vi "Open Deployed Project.vi"() -> ()   [LabVIEW 2023]
doc: "Tools >> Systemcore >> Open Deployed Project: copies the program a robot runs (its current deploy) into a git working copy on the robot-edits branch and opens its LabVIEW project. When the robot keeps several projects, the user chooses one. In the robot's own IDE it uses ~/Projects/<project name> (reusing an existing copy); on a desktop it asks for the robot's address and a new folder."
uses:
  <vilib>/Utility/sysdir.llb/System Directory Type.ctl
panel:
  out "Status":string
types:
  T1 = typedef "System Directory Type.ctl" = i32
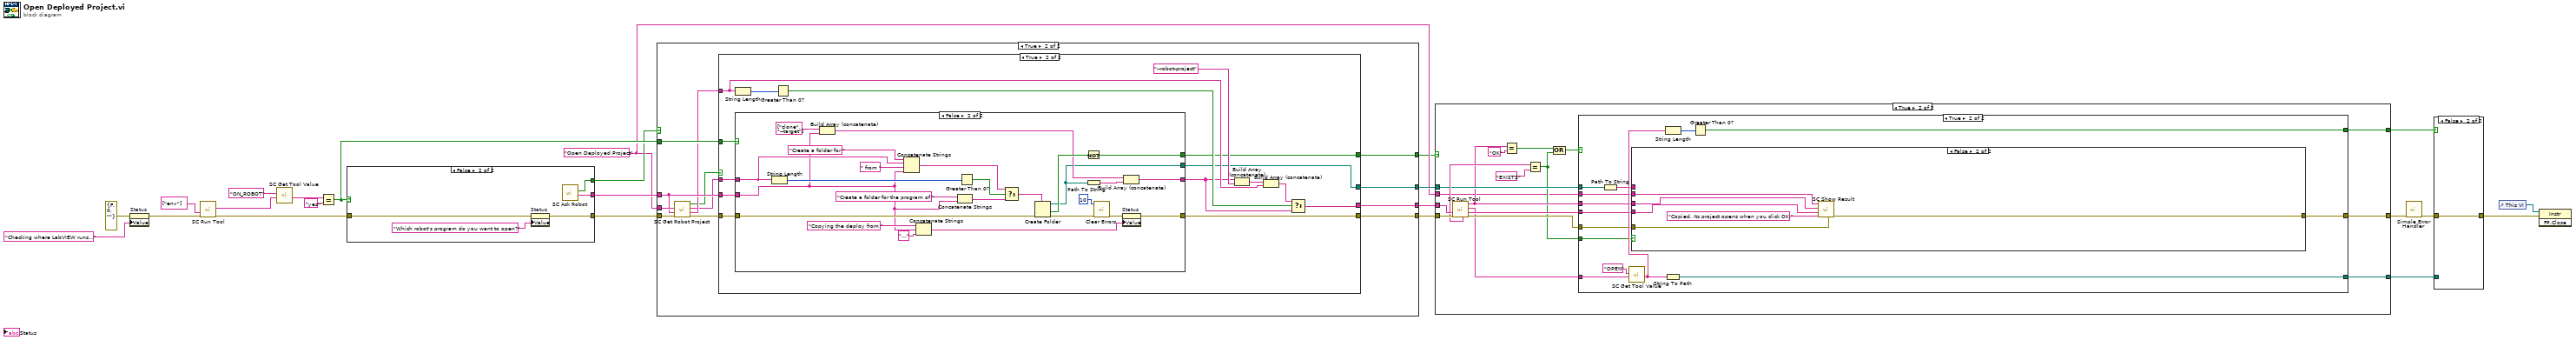
[diagram p0: block diagram]
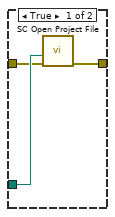
[diagram p2: hidden frame]
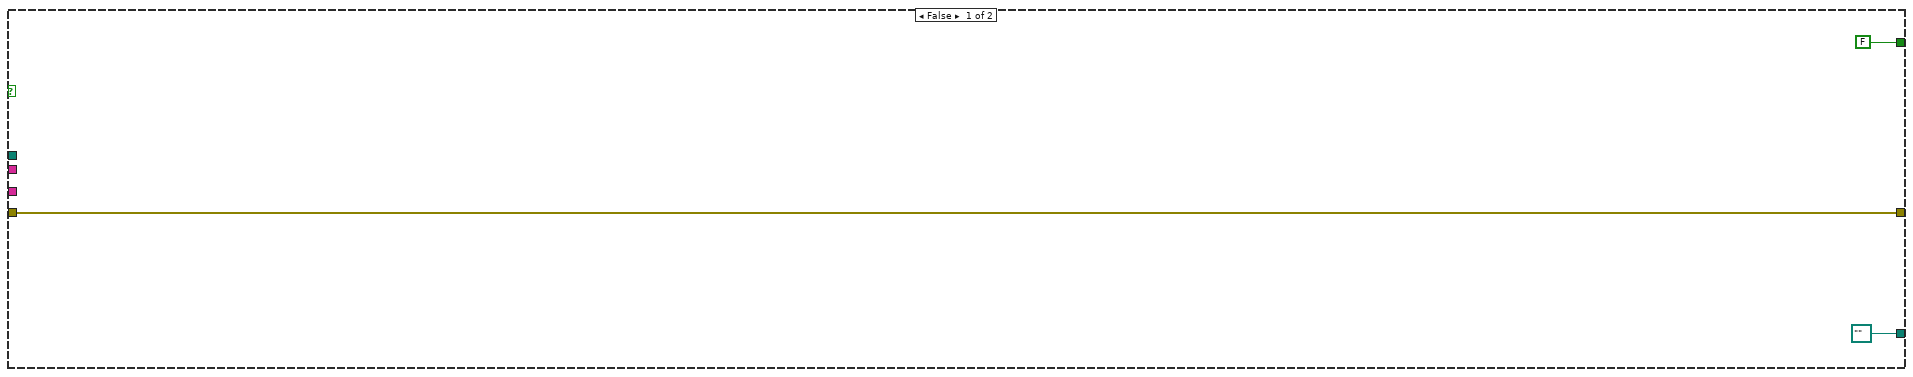
[diagram p3: hidden frame]
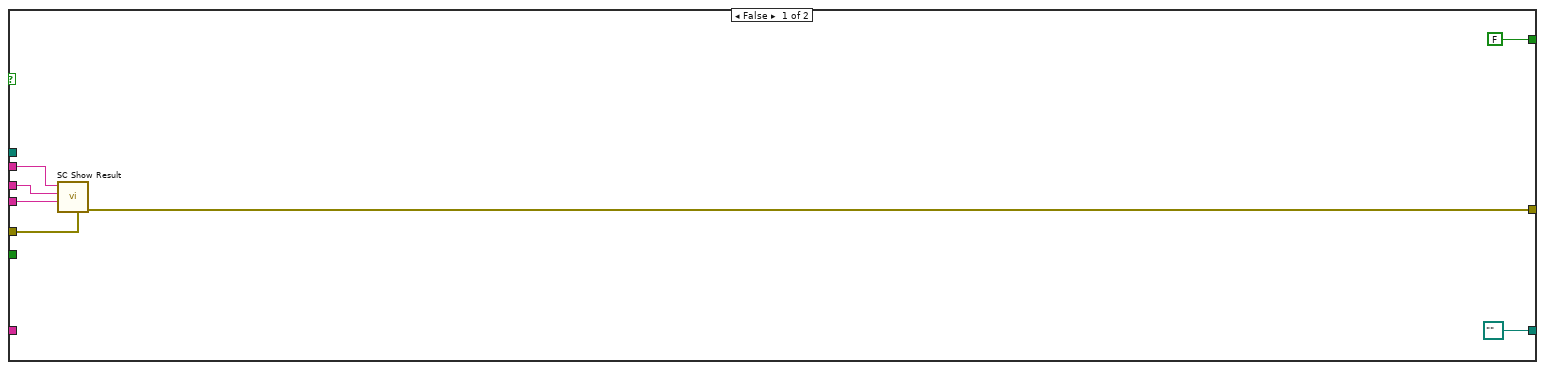
[diagram p4: hidden frame]
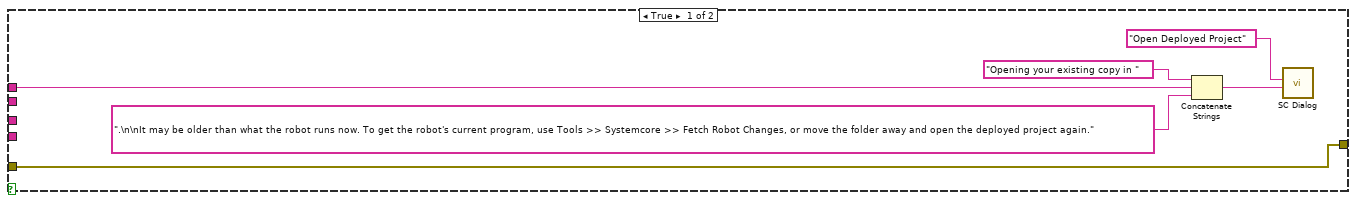
[diagram p5: hidden frame]
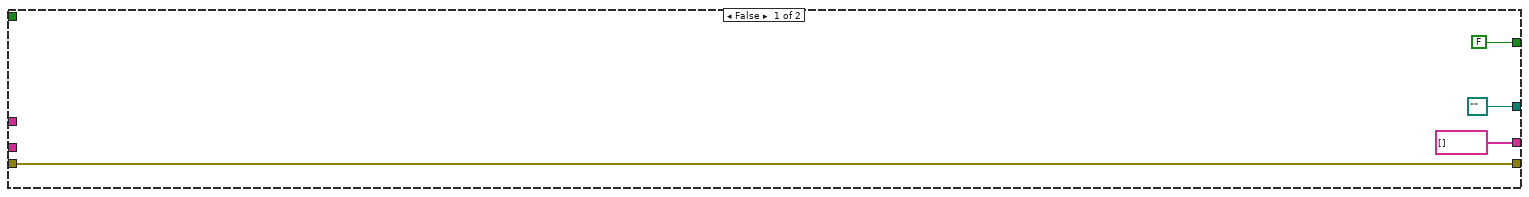
[diagram p6: hidden frame]
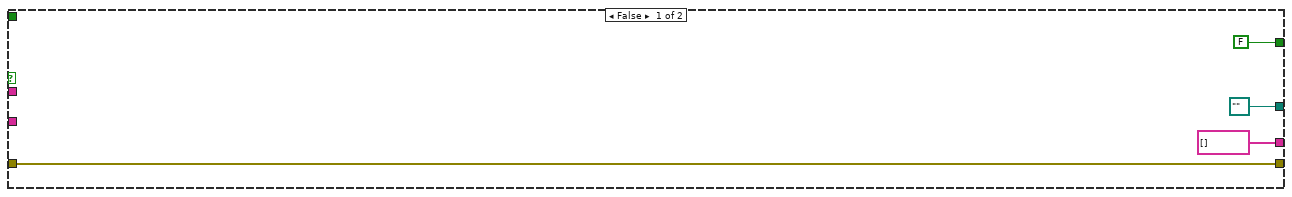
[diagram p7: hidden frame]
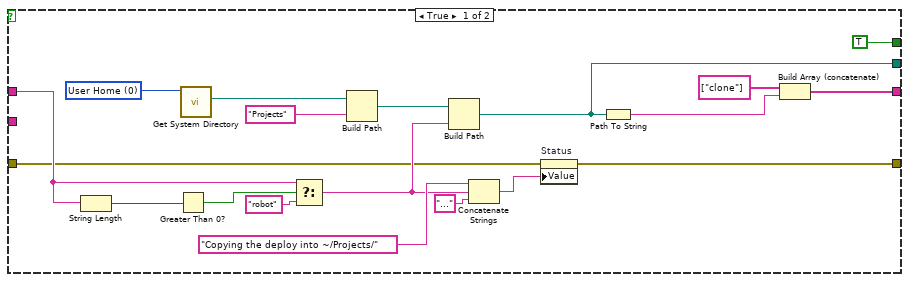
[diagram p8: hidden frame]
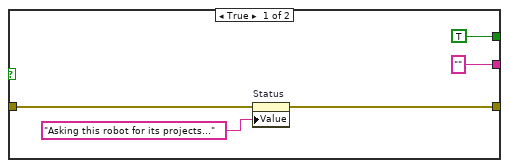
[diagram p9: hidden frame]
diagram:
  w8 = "Open Deployed Project"
  n1 = property on="Status" class="Str"(error in=errorcluster {"status"=FALSE, "code"=0, "source"=""}, "Value"="Checking where LabVIEW runs...") -> (error out=w21:errorcluster)  [unwired: 1 in, 1 out]
  n2 = call "SC Run Tool.vi"("error in (no error)"=w21, "arguments"=string[] ["env"]) -> ("error out"=w16:errorcluster, "tool lines"=w20:string[])  [unwired: 4 in, 4 out]
  n3 = call "SC Get Tool Value.vi"("tool lines"=w20, "key"="ON_ROBOT") -> ("value"=w18:string)  [unwired: 8 in, 1 out]
  n4 = Equal?(x=w18, y="yes") -> (x = y?=w13:bool)
  n5 = case shown="False" w13 {
    tunnel: w16 -> [w29 w34]
    tunnel: [TRUE w32] -> w12
    tunnel: ["" w31] -> w15
    tunnel: [w25 w30] -> w14
    frame True {
      n6 = property on="Status" class="Str"(error in=w29, "Value"="Asking this robot for its projects...") -> (error out=w25:errorcluster)  [unwired: 1 in, 1 out]
    }
    frame False {
      n7 = property on="Status" class="Str"(error in=w34, "Value"="Which robot's program do you want to open?") -> (error out=w30:errorcluster)  [unwired: 1 in, 1 out]
      n8 = call <vilib>:"SC Ask Robot.vi"() -> ("address"=w31:string, "ok?"=w32:bool)  [unwired: 10 in]
    }
  }
  n9 = case shown="True" w12 {
    tunnel: w15 -> [_ w48]
    tunnel: w14 -> [w35 w49]
    tunnel: w8 -> [_ w50]
    tunnel: w13 -> [_ w46]
    tunnel: [FALSE w42] -> w7
    tunnel: [string[] [] w41] -> w11
    tunnel: [path "" w40] -> w10
    tunnel: [w35 w39] -> w9
    frame False {
    }
    frame True {
      n10 = call "SC Get Robot Project.vi"("error in (no error)"=w49, "target"=w48, "window title"=w50) -> ("error out"=w47:errorcluster, "root"=w45:string, "name"=w44:string, "chosen?"=w43:bool)  [unwired: 5 in]
      n11 = case shown="True" w43 {
        tunnel: w48 -> [_ w69]
        tunnel: w47 -> [w51 w68]
        tunnel: w46 -> [_ w66]
        tunnel: w45 -> [_ w63]
        tunnel: w44 -> [_ w67]
        tunnel: [FALSE w58] -> w42
        tunnel: [string[] [] w57] -> w41
        tunnel: [path "" w56] -> w40
        tunnel: [w51 w55] -> w39
        frame False {
        }
        frame True {
          n12 = String Length(string=w63) -> (length=w62:i32)
          n13 = case shown="False" w66 {
            tunnel: w69 -> [_ w96]
            tunnel: w68 -> [w75 w105]
            tunnel: w67 -> [w86 w110]
            tunnel: [TRUE w92] -> w58
            tunnel: [w72 w91] -> w59
            tunnel: [w71 w90] -> w56
            tunnel: [w70 w89] -> w55
            frame True {
              w84 = T1 0 items=["User Home"=0, "User Desktop"=1, "User Documents"=2, "User Application Data"=3, "User Preferences"=4, "User Temporary"=5, "Public Documents"=6, "Public Application Data"=7, "Public Preferences"=8, "Public Cache"=13, "System Core Libraries"=9, "System Installed Libraries"=10, "Application Files"=11, "Boot Volume Root"=12]
              n14 = String Length(string=w86) -> (length=w88:i32)
              n15 = Greater Than 0?(x=w88) -> (x > 0?=w87:bool)
              n16 = call <vilib>:"Get System Directory.vi"("system directory type"=w84) -> ("system directory"=w83:path)  [unwired: 10 in]
              n17 = Select(t=w86, s=w87, f="robot") -> (s? t:f=w77:string)
              n18 = Build Path(base path=w83, name or relative path="Projects") -> (appended path=w81:path)
              n19 = Build Path(base path=w81, name or relative path=w77) -> (appended path=w71:path)
              n20 = Concatenate Strings("Copying the deploy into ~/Projects/", w77, "...") -> (w74:string)
              n21 = property on="Status" class="Str"(error in=w75, "Value"=w74) -> (error out=w70:errorcluster)  [unwired: 1 in, 1 out]
              n22 = Path To String(path=w71) -> (string=w79:string)
              n23 = Build Array (concatenate)(string[] ["clone"], w79) -> (w72:string[])
            }
            frame False {
              n24 = String Length(string=w110) -> (length=w109:i32)
              n25 = Build Array (concatenate)(string[] ["clone", "--target"], w96) -> (w99:string[])
              n26 = Concatenate Strings("Create a folder for ", w110, " from ", w96) -> (w107:string)
              n27 = Concatenate Strings("Copying the deploy from ", w96, "...") -> (w93:string)
              n28 = Concatenate Strings("Create a folder for the program of ", w96) -> (w106:string)
              n29 = Greater Than 0?(x=w109) -> (x > 0?=w108:bool)
              n30 = Select(t=w107, s=w108, f=w106) -> (s? t:f=w104:string)
              n31 = Create Folder(prompt (Create Folder)=w104, error in=w105) -> (created path=w90:path, cancelled=w101:bool, error out=w103:errorcluster)  [unwired: 1 in]
              n32 = Not(x=w101) -> (.not. x?=w92:bool)
              n33 = Path To String(path=w90) -> (string=w98:string)
              n34 = call <vilib>:"Clear Errors.vi"("error in (no error)"=w103, "specific error code to clear (0: all)"=10) -> ("error out"=w94:errorcluster)  [unwired: 4 in, 1 out]
              n35 = property on="Status" class="Str"(error in=w94, "Value"=w93) -> (error out=w89:errorcluster)  [unwired: 1 in, 1 out]
              n36 = Build Array (concatenate)(w99, w98) -> (w91:string[])
            }
          }
          n37 = Greater Than 0?(x=w62) -> (x > 0?=w61:bool)
          n38 = Build Array (concatenate)(w59, "--robot-project") -> (w64:string[])
          n39 = Build Array (concatenate)(w64, w63) -> (w60:string[])
          n40 = Select(t=w60, s=w61, f=w59) -> (s? t:f=w57:string[])
        }
      }
    }
  }
  n41 = case shown="True" w7 {
    tunnel: w11 -> [_ w133]
    tunnel: w10 -> [_ w127]
    tunnel: w9 -> [w116 w132]
    tunnel: w8 -> [_ w122]
    tunnel: [w116 w119] -> w6
    tunnel: [path "" w118] -> w5
    tunnel: [FALSE w117] -> w3
    frame False {
    }
    frame True {
      n42 = call "SC Run Tool.vi"("error in (no error)"=w132, "arguments"=w133) -> ("error out"=w126:errorcluster, "output"=w125:string, "tool lines"=w121:string[], "result"=w124:string, "result detail"=w130:string)  [unwired: 4 in, 1 out]
      n43 = Equal?(x=w124, y="OK") -> (x = y?=w128:bool)
      n44 = Equal?(x=w130, y="EXISTS") -> (x = y?=w123:bool)
      n45 = Compound Arithmetic op=OR(w128, w123) -> (w120:bool)
      n46 = case shown="True" w120 {
        tunnel: w127 -> [_ w150]
        tunnel: w126 -> [w137 w148]
        tunnel: w125 -> [w140 w147]
        tunnel: w124 -> [w139 w146]
        tunnel: w123 -> [_ w144]
        tunnel: w122 -> [w138 w145]
        tunnel: w121 -> [_ w154]
        tunnel: [w136 w143] -> w119
        tunnel: [path "" w142] -> w118
        tunnel: [FALSE w141] -> w117
        frame False {
          n47 = call "SC Show Result.vi"("error in (no error)"=w137, "output"=w140, "result"=w139, "title"=w138) -> ("error out"=w136:errorcluster)  [unwired: 7 in]
        }
        frame True {
          n48 = Path To String(path=w150) -> (string=w149:string)
          n49 = call "SC Get Tool Value.vi"("tool lines"=w154, "key"="OPEN") -> ("value"=w152:string)  [unwired: 8 in, 1 out]
          n50 = case shown="False" w144 {
            tunnel: w149 -> [w159 _]
            tunnel: w148 -> [w155 w162]
            tunnel: w147 -> [_ w166]
            tunnel: w146 -> [_ w165]
            tunnel: w145 -> [_ w164]
            tunnel: [w155 w161] -> w143
            frame True {
              n51 = Concatenate Strings("Opening your existing copy in ", w159, ".\n\nIt may be older than what the robot runs now. To get the robot's current program, use Tools >> Systemcore >> Fetch Robot Changes, or move the folder away and open the deployed project again.") -> (w157:string)
              n52 = call "SC Dialog.vi"("message"=w157, "window title"="Open Deployed Project") -> ()  [unwired: 9 in, 1 out]
            }
            frame False {
              n53 = call "SC Show Result.vi"("error in (no error)"=w162, "OK message"="Copied. Its project opens when you click OK.", "output"=w166, "result"=w165, "title"=w164) -> ("error out"=w161:errorcluster)  [unwired: 6 in]
            }
          }
          n54 = String To Path(string=w152) -> (path=w142:path)
          n55 = String Length(string=w152) -> (length=w151:i32)
          n56 = Greater Than 0?(x=w151) -> (x > 0?=w141:bool)
        }
      }
    }
  }
  n57 = call <vilib>:"Simple Error Handler.vi"("error in (no error)"=w6) -> ("error out"=w4:errorcluster)  [unwired: 4 in, 4 out]
  n58 = case shown="False" w3 {
    tunnel: w5 -> [w169 _]
    tunnel: w4 -> [w168 w170]
    tunnel: [w167 w170] -> w1
    frame True {
      n59 = call "SC Open Project File.vi"("error in (no error)"=w168, "path"=w169) -> ("error out"=w167:errorcluster)  [unwired: 9 in]
    }
    frame False {
    }
  }
  n60 = control-ref of="This VI"() -> (w2:refnum<vi>)
  n61 = invoke class="Instr" method="FP.Close"(reference=w2, error in=w1) -> ()  [unwired: 1 in, 3 out]
